vi "Test - Day Total Entries Cases.vi"(8 "error in":errorcluster, 10 "Work Folder":path, 11 "Test Data Folder":path) -> (0 "error out":errorcluster, 3 "Conditions":bool[](array[boolean]))   [LabVIEW 2026]
doc: "Test support for Test Day Total.vi. Copies Test Data\\Samples into a new case folder, adds three entries through the Time Entry Store (DT-CROSS 2025-10-14 22:30 to 2025-10-15 01:30, DT-MONTH 2025-10-31 18:30 to 2025-11-01 00:30 - filed in the October file, DT-DST 2026-03-09 00:30 to 00:45 - on the day after the 23-hour day), then runs Day Total Entries.vi and Day Total.vi for 2025-10-15, 2025-11-01, 2025-11-04, 2025-11-03 and 2026-03-09 (local times, US Central). Conditions holds ten results in this order: the five days' Total Entries IDs (joined with ;) as expected, then the five days' Total Text as expected.\n\nInputs: Test Data Folder; Work Folder; error in. Outputs: Conditions; error out.\n\nGenerated by: Claude"
uses:
  Storage/Time Entry Store/Time Entry Store.lvclass
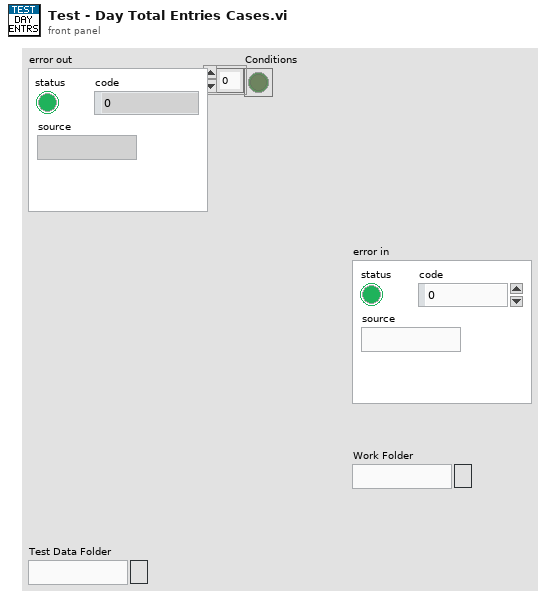
[diagram p1: front panel]
types:
  T1 = cluster{"ID":string, "Project ID":string, "Task ID":string, "Start Time":timestamp, "End Time":timestamp, "Description":string}
  T2 = typedef "Time Entry List.ctl" = T3[]
  T3 = typedef "Time Entry.ctl" = cluster{"ID":string, "Project ID":string, "Task ID":string, "Start Time":timestamp, "End Time":timestamp, "Description":string}
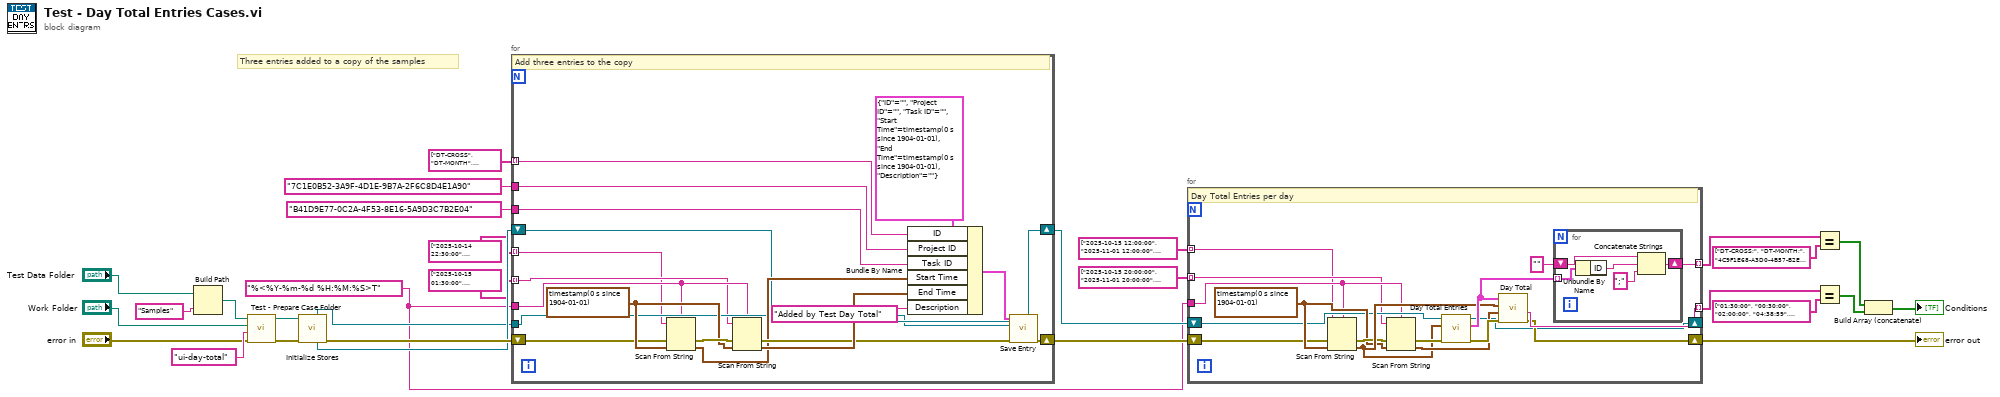
[diagram p0: block diagram]
diagram:
  w6 = "%<%Y-%m-%d %H:%M:%S>T" ("local time format")
  # "Three entries added to a copy of the samples"
  n1 = Build Path(base path="Test Data Folder", name or relative path="Samples" ("samples")) -> (appended path=w18:path)
  n2 = call "Test - Prepare Case Folder.vi"("error in (no error)"="error in", "Case Name"="ui-day-total" ("case name"), "Work Folder"="Work Folder", "Source Folder"=w18) -> ("error out"=w20:errorcluster, "Case Folder"=w19:path)  [unwired: 6 in]
  n3 = call "Initialize Stores.vi"("error in"=w20, "Data Folder"=w19) -> ("error out"=w23:errorcluster, "Time Entry Store out"=w22:refnum<class "Time Entry Store.lvclass">, "Project Store out"=w21:refnum<class "Project Store.lvclass">)  [unwired: 5 in, 2 out]
  n4 = for {
    tunnel: string[] ["DT-CROSS", "DT-MONTH", "DT-DST"] ("added IDs") -> [w30] mode=indexing
    tunnel: string[] ["2025-10-14 22:30:00", "2025-10-31 18:30:00", "2026-03-09 00:30:00"] ("added starts") -> [w31] mode=indexing
    tunnel: string[] ["2025-10-15 01:30:00", "2025-11-01 00:30:00", "2026-03-09 00:45:00"] ("added ends") -> [w32] mode=indexing
    tunnel: w6 -> [w33]
    tunnel: "7C1E0B52-3A9F-4D1E-9B7A-2F6C8D4E1A90" ("added Project ID") -> [w34]
    tunnel: "B41D9E77-0C2A-4F53-8E16-5A9D3C7B2E04" ("added Task ID") -> [w35]
    tunnel: w21 -> [w36]
    shift-right: [w38] -> w24
    shift-left: w22 -> [w37]
    shift-right: [w40] -> w25
    shift-left: w23 -> [w39]
    w42 = timestamp(0 s since 1904-01-01) ("default time")
    # "Add three entries to the copy"
    n5 = Scan From String(format string=w33, input string=w31, error in=w39, default 1=w42) -> (error out=w44:errorcluster, output 1=w45:timestamp)  [unwired: 1 in, 2 out]
    n6 = Scan From String(format string=w33, input string=w32, error in=w44, default 1=w42) -> (error out=w46:errorcluster, output 1=w47:timestamp)  [unwired: 1 in, 2 out]
    n7 = Bundle By Name(cluster=T1 {"ID"="", "Project ID"="", "Task ID"="", "Start Time"=timestamp(0 s since 1904-01-01), "End Time"=timestamp(0 s since 1904-01-01), "Description"=""} ("entry"), "ID"=w30, "Project ID"=w34, "Task ID"=w35, "Start Time"=w45, "End Time"=w47, "Description"="Added by Test Day Total") -> (w48:T1)
    n8 = call-dynamic "Save Entry.vi"("Time Entry Store in"=w37, "error in (no error)"=w46, "Project Store"=w36, "Time Entry"=w48) -> ("error out"=w40:errorcluster, "Time Entry Store out"=w38:refnum<class "Time Entry Store.lvclass">)  [unwired: 6 in]
  }
  n9 = for {
    tunnel: string[] ["2025-10-15 12:00:00", "2025-11-01 12:00:00", "2025-11-04 12:00:00", "2025-11-03 12:00:00", "2026-03-09 12:00:00"] ("store days") -> [w49] mode=indexing
    tunnel: string[] ["2025-10-15 20:00:00", "2025-11-01 20:00:00", "2025-11-04 02:00:00", "2025-11-03 12:00:00", "2026-03-09 20:00:00"] ("store nows") -> [w50] mode=indexing
    tunnel: w6 -> [w51]
    tunnel: [w65] -> w26 mode=indexing
    shift-right: [w53] -> _
    shift-left: w24 -> [w52]
    shift-right: [w55] -> w5
    shift-left: w25 -> [w54]
    tunnel: [w64] -> w27 mode=indexing
    w56 = timestamp(0 s since 1904-01-01) ("default time")
    # "Day Total Entries per day"
    n10 = Scan From String(format string=w51, input string=w49, error in=w54, default 1=w56) -> (error out=w58:errorcluster, output 1=w59:timestamp)  [unwired: 1 in, 2 out]
    n11 = Scan From String(format string=w51, input string=w50, error in=w58, default 1=w56) -> (error out=w60:errorcluster, output 1=w61:timestamp)  [unwired: 1 in, 2 out]
    n12 = call "Day Total Entries.vi"("error in"=w60, "Day"=w59, "Time Entry Store in"=w52) -> ("error out"=w63:errorcluster, "Total Entries"=w62:T2, "Time Entry Store out"=w53:refnum<class "Time Entry Store.lvclass">)  [unwired: 6 in]
    n13 = call "Day Total.vi"("error in"=w63, "Now"=w61, "Day"=w59, "Entries"=w62) -> ("error out"=w55:errorcluster, "Total Text"=w64:string)  [unwired: 5 in, 1 out]
    n14 = for {
      shift-right: [w68] -> w65
      shift-left: "" ("no IDs") -> [w67]
      tunnel: w62 -> [w66] mode=indexing
      n15 = Unbundle By Name(w66) -> ("ID"=w70:string)
      n16 = Concatenate Strings(w67, w70, ";" ("separator")) -> (w68:string)
    }
  }
  "error out" <- w5
  n17 = Equal?(x=w26, y=string[] ["DT-CROSS;", "DT-MONTH;", "4C9F1E68-A3D0-4B57-B2E9-6A0C8D5F3B71;", "E7A30D5C-2B84-4F19-8C6A-9D1E4B7F0A32;4C9F1E68-A3D0-4B57-B2E9-6A0C8D5F3B71;", "DT-DST;"] ("expected IDs")) -> (x = y?=w28:bool[])
  n18 = Equal?(x=w27, y=string[] ["01:30:00", "00:30:00", "02:00:00", "04:38:59", "00:15:00"] ("expected day texts")) -> (x = y?=w29:bool[])
  n19 = Build Array (concatenate)(w28, w29) -> (→"Conditions":bool[])
